vi "UBX GPS Decode (sim) Example.vi"() -> ()   [LabVIEW 2015]
panel:
  out "CK_B":u8 format="%02x"
  out "CK_A":u8 format="%02x"
  out "size(s)":i32
  out "Payload":u8[](array[numeric]) format="%02x"
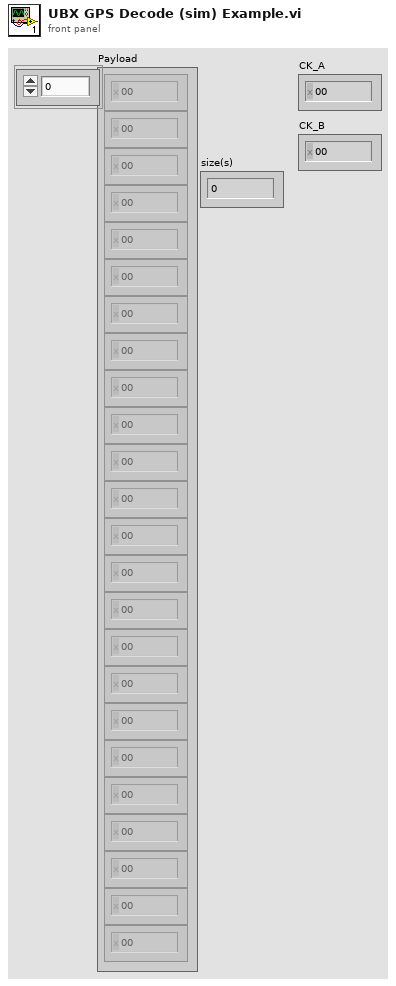
[diagram p1: front panel]
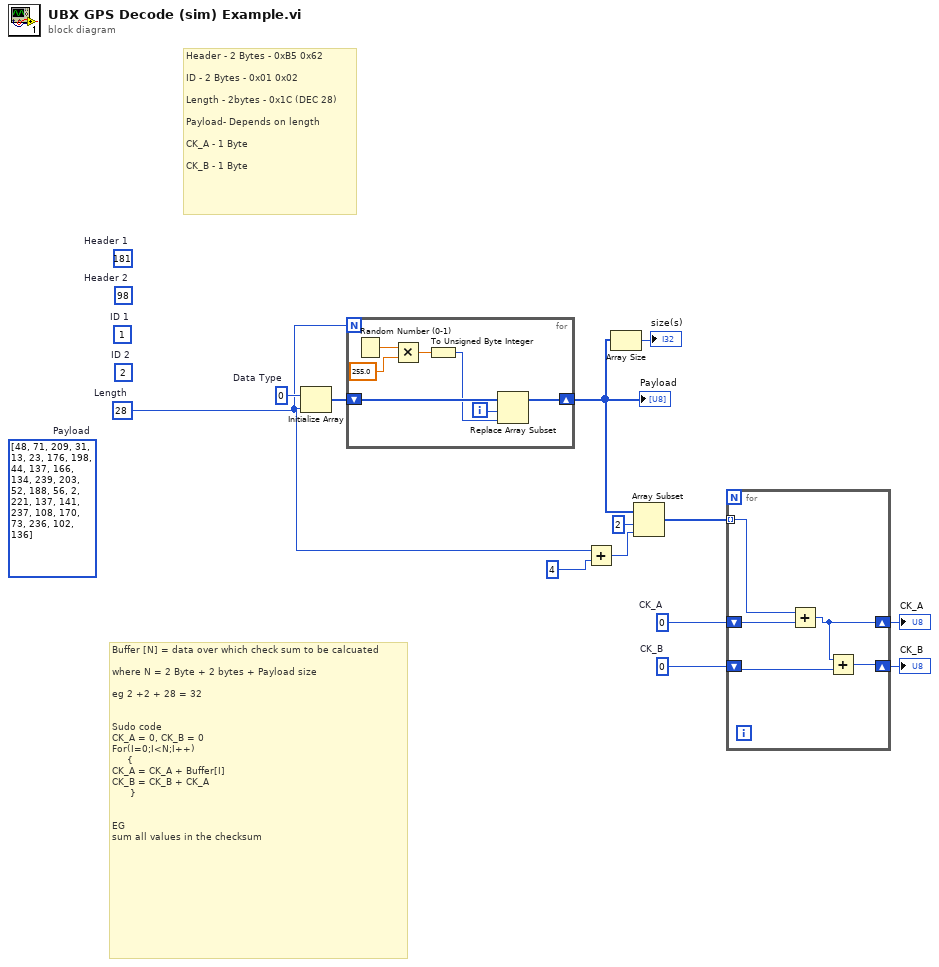
[diagram p0: block diagram]
diagram:
  w3 = 0  # CK_B
  w4 = 0  # CK_A
  (unwired) u8[] [48, 71, 209, 31, 13, 23, 176, 198, 44, 137, 166, 134, 239, 203, 52, 188, 56, 2, 221, 137, 141, 237, 108, 170, 73, 236, 102, 136]  # Payload
  w7 = u8 28  # Length
  (unwired) u8 2  # ID 2
  (unwired) u8 1  # ID 1
  (unwired) u8 98  # Header 2
  (unwired) u8 181  # Header 1
  w13 = u8 0  # Data Type
  # "Buffer [N] = data over which check sum to be calcuated\n\nwhere N = 2 Byte + 2 bytes + Payload size\n\neg 2 +2 + 28 = 32\n\n\nSudo code\nCK_A = 0, CK_B = 0\nFor(I=0;I<N;I++)\n     {\nCK_A = CK_A + Buffer[I]\nCK_B = CK_B + CK_A\n      }\n\n\nEG\nsum all values in the checksum"
  # "Header - 2 Bytes - 0xB5 0x62\n\nID - 2 Bytes - 0x01 0x02\n\nLength - 2bytes - 0x1C (DEC 28) \n\nPayload- Depends on length\n\nCK_A - 1 Byte\n\nCK_B - 1 Byte"
  n1 = Initialize Array(w13, w7) -> (w12:u8[])
  n2 = for {
    N: w7 -> [_]
    shift-right: [w14] -> w10
    shift-left: w12 -> [w20]
    i -> [w15]
    n3 = Random Number (0-1)() -> (number: 0 to 1=w17:dbl)
    n4 = Multiply(x=w17, y=255.0) -> (x*y=w19:dbl)
    n5 = To Unsigned Byte Integer(number=w19) -> (unsigned 8bit integer=w16:u8)
    n6 = Replace Array Subset(array=w20, new element=w16, index=w15) -> (w14:u8[])
  }
  "Payload" <- w10
  n7 = Add(x=w7, y=4 ("index")) -> (x+y=w6:i32)
  n8 = Array Size(array=w10) -> (size(s)=→"size(s)":i32)
  n9 = Array Subset(array=w10, index=2, length=w6) -> (w5:u8[])
  n10 = for {
    tunnel: w5 -> [w24] mode=indexing
    shift-right: [w22] -> w2
    shift-left: w4 -> [w25]
    shift-right: [w23] -> w1
    shift-left: w3 -> [w21]
    n11 = Add(x=w24, y=w25) -> (x+y=w22:i32)
    n12 = Add(x=w22, y=w21) -> (x+y=w23:i32)
  }
  "CK_A" <- w2
  "CK_B" <- w1
